vi "DumpFileInit.vi"() -> (3 "DumpFileQueue":T1)   [LabVIEW 2018]
uses:
  DumpFileQueue.ctl
  DumpFileEvent.ctl
  DumpFileAction.ctl
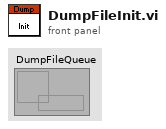
[diagram p1: front panel]
types:
  T1 = typedef "DumpFileQueue.ctl" = refnum<queue>
  T2 = typedef "DumpFileEvent.ctl" = cluster{"Path":path, "DumpFileAction":T3, "Data":dbl[][]}
  T3 = typedef "DumpFileAction.ctl" = enum16{"StartNew", "StartAppend", "Data", "Close"}
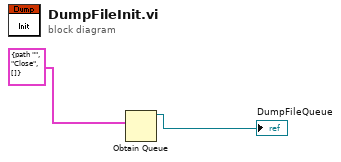
[diagram p0: block diagram]
diagram:
  n1 = Obtain Queue(element data type=T2 {"Path"=path "", "DumpFileAction"=enum."Close", "Data"=[]} ("DumpFileEvent")) -> (queue out=→"DumpFileQueue":refnum<queue>)  [unwired: 4 in, 2 out]
